vi "Remove Last Item from Peek Stack.vi"(8 "error in (no error)":errorcluster, 11 "Data Cluster in":T1={"PeekVI Reference"=refnum, "SubPanel"=refnum, "Peek Stack Tree Ref"=refnum, "Open Button Ref"=refnum, "Top VI"=refnum, "Active VI"=refnum, "Stack"=[], "Last FP State"=enum."Standard"}) -> (0 "error out":errorcluster, 2 "Removed VI":refnum<class "Standard VI Type.lvclass">, 3 "Data Cluster out":T1={"PeekVI Reference"=refnum, "SubPanel"=refnum, "Peek Stack Tree Ref"=refnum, "Open Button Ref"=refnum, "Top VI"=refnum, "Active VI"=refnum, "Stack"=[], "Last FP State"=enum."Standard"})   [LabVIEW 2020, in "Peek Window.lvlib"]
uses:
  Peek Window.lvlib
  MHL Data Cluster.ctl
  VI Types/Standard VI Type/Standard VI Type.lvclass
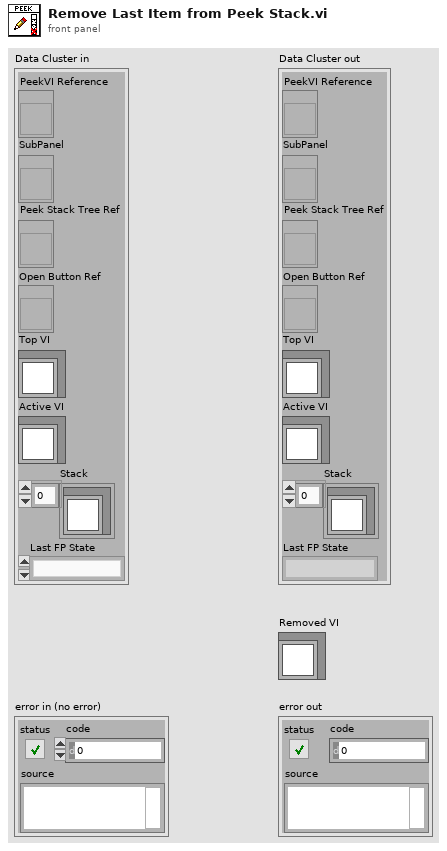
[diagram p1: front panel]
types:
  T1 = typedef "Peek Window.lvlib/MHL Data Cluster.ctl" = cluster{"PeekVI Reference":refnum<vi>, "SubPanel":refnum<vi>, "Peek Stack Tree Ref":refnum<vi>, "Open Button Ref":refnum<vi>, "Top VI":refnum<class "Standard VI Type.lvclass">, "Active VI":refnum<class "Standard VI Type.lvclass">, "Stack":refnum<class "Standard VI Type.lvclass">[], "Last FP State":enum32{"Invalid", "Standard", "Closed", "Hidden", "Minimized", "Maximized"}}
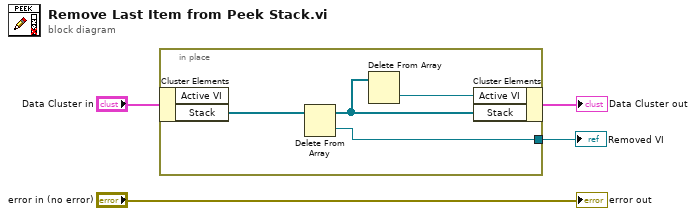
[diagram p0: block diagram]
diagram:
  n1 = in-place {
    in-place-border: [w8] -> w1
    n2 = in-place-cluster #1("Data Cluster in") -> ("Stack"=w5:refnum<class "Standard VI Type.lvclass">[])  [unwired: 1 out]
    n3 = Delete From Array(array=w5) -> (deleted portion=w8:refnum<class "Standard VI Type.lvclass">, array with subset deleted=w7:refnum<class "Standard VI Type.lvclass">[])  [unwired: 2 in]
    n4 = Delete From Array(array=w7) -> (deleted portion=w6:refnum<class "Standard VI Type.lvclass">)  [unwired: 2 in, 1 out]
    n5 = in-place-cluster #1("Active VI"=w6, "Stack"=w7) -> (→"Data Cluster out":T1)
  }
  "Removed VI" <- w1
  "error out" <- "error in (no error)"
